vi "IR ini file creation.vi"(0 "IR Test Time(S)":string, 1 "IR voltage(kV)":string, 2 "configuration file path":path, 5 "IR LO SET":string, 7 "IR HI SET":string, 9 "Ramp Time":string, 11 "error in (no error) 2":errorcluster) -> (15 "error in (no error) 3":errorcluster)   [LabVIEW 2021]
uses:
  Template/Main_VI/Control/Ini.ctl
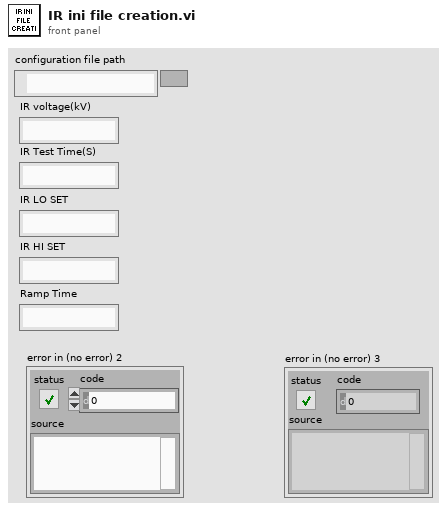
[diagram p1: front panel]
types:
  T1 = typedef "Ini.ctl" = enum16{"Write", "Read"}
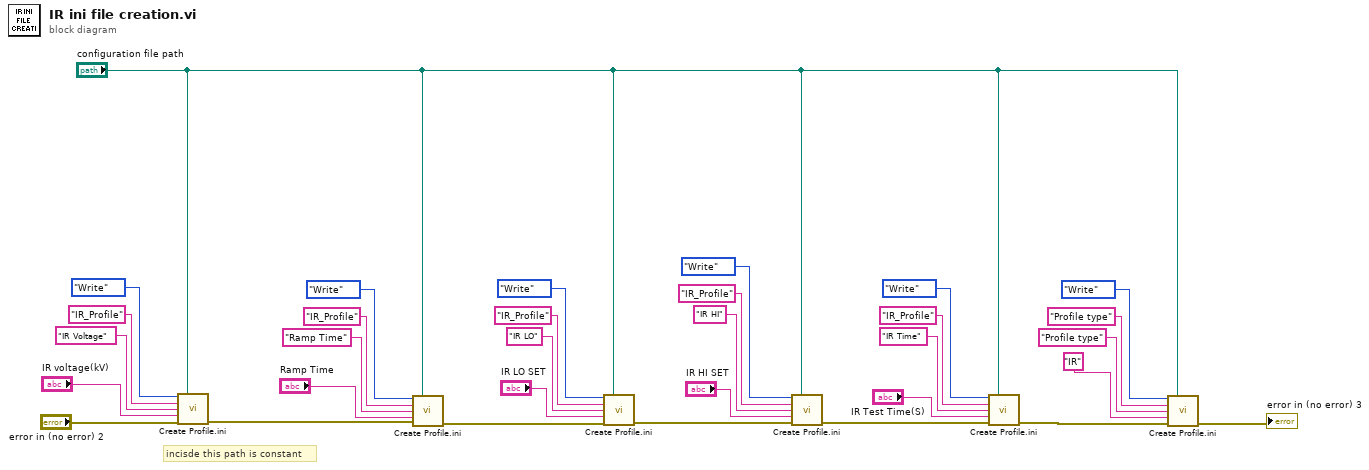
[diagram p0: block diagram]
diagram:
  # "incisde this path is constant"
  n1 = call "Create Profile.ini.vi"(0:Ini."Write", "configuration file path"="configuration file path", "Write Section"="IR_Profile", "Write key"="IR Voltage", "Write"="IR voltage(kV)", "error in (no error)"="error in (no error) 2") -> ("error in (no error) 3"=w17:errorcluster)  [unwired: 8 in, 1 out]
  n2 = call "Create Profile.ini.vi"(0:Ini."Write", "configuration file path"="configuration file path", "Write Section"="IR_Profile", "Write key"="Ramp Time", "Write"="Ramp Time", "error in (no error)"=w17) -> ("error in (no error) 3"=w16:errorcluster)  [unwired: 8 in, 1 out]
  n3 = call "Create Profile.ini.vi"(0:Ini."Write", "configuration file path"="configuration file path", "Write Section"="IR_Profile", "Write key"="IR LO", "Write"="IR LO SET", "error in (no error)"=w16) -> ("error in (no error) 3"=w15:errorcluster)  [unwired: 8 in, 1 out]
  n4 = call "Create Profile.ini.vi"(0:Ini."Write", "configuration file path"="configuration file path", "Write Section"="IR_Profile", "Write key"="IR HI", "Write"="IR HI SET", "error in (no error)"=w15) -> ("error in (no error) 3"=w14:errorcluster)  [unwired: 8 in, 1 out]
  n5 = call "Create Profile.ini.vi"(0:Ini."Write", "configuration file path"="configuration file path", "Write Section"="IR_Profile", "Write key"="IR Time", "Write"="IR Test Time(S)", "error in (no error)"=w14) -> ("error in (no error) 3"=w8:errorcluster)  [unwired: 8 in, 1 out]
  n6 = call "Create Profile.ini.vi"(0:Ini."Write", "configuration file path"="configuration file path", "Write Section"="Profile type", "Write key"="Profile type", "Write"="IR", "error in (no error)"=w8) -> ("error in (no error) 3"=→"error in (no error) 3":errorcluster)  [unwired: 8 in, 1 out]
